vi "Create.vi"(8 "error in (no error)":errorcluster, 11 "Templates Root":path) -> (0 "error out":errorcluster, 3 "BasicTemplater out":refnum<class "BasicTemplater.lvclass">)   [LabVIEW 2020, in "HTTP Server.lvlib" / "BasicTemplater.lvclass"]
uses:
  BasicTemplater.lvclass
  BasicTemplater.lvclass/BasicTemplater.ctl
  TemplateVariableResolver/TemplateValueResolver.lvclass
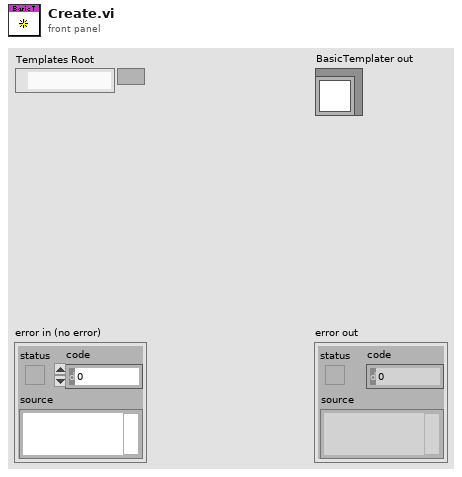
[diagram p1: front panel]
types:
  T1 = map{string, refnum<class "TemplateValueResolver.lvclass">}
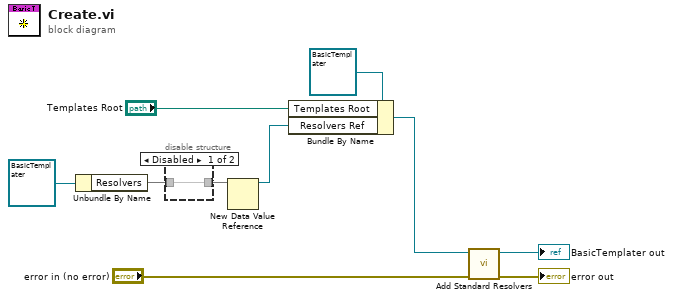
[diagram p0: block diagram]
diagram:
  n1 = Unbundle By Name(refnum<class "BasicTemplater.lvclass"> refnum ("BasicTemplater in")) -> ("Resolvers"=w6:T1)
  n2 = disable-structure shown="Disabled" {
    disable-tunnel: [w11 _] -> w7
    disable-tunnel: w6 -> [w11 _]
    frame Disabled {
    }
    frame Enabled {
    }
  }
  n3 = New Data Value Reference(data value=w7) -> (data value reference=w5:refnum<data-value>)  [unwired: 1 in, 1 out]
  n4 = Bundle By Name(cluster=refnum<class "BasicTemplater.lvclass"> refnum ("BasicTemplater in"), "Templates Root"="Templates Root", "Resolvers Ref"=w5) -> (w9:refnum<class "BasicTemplater.lvclass">)
  n5 = call "Add Standard Resolvers.vi"("error in (no error)"="error in (no error)", "BasicTemplater in"=w9) -> ("error out"=→"error out":errorcluster, "BasicTemplater out"=→"BasicTemplater out":refnum<class "BasicTemplater.lvclass">)  [unwired: 8 in]
